vi "ASD total S analysis.vi"(4 "AF_C":cluster{"Anal Time":string, "Filename":string}, 5 "1s datapoint":i32, 6 "Read Region Point":i32=10000, 7 "B Region Time [s] in":dbl, 8 "Rigon#":i32, 9 "Region Count":dbl[](array[numeric]), 10 "Region STD":dbl[](array[numeric]), 11 "Region BL":dbl[](array[numeric])) -> (3 "A Cluster":T1)   [LabVIEW 2018]
uses:
  <vilib>/Analysis/baseanly.llb/Unimode.vi
  <vilib>/Analysis/NI_AALBase.lvlib
panel:
  out "B Duty Cycle [%]":dbl
  out "Total Time [s]":dbl
  out "Region Count Mode":dbl caption="R Count Mode [a]"
  out "Region BL Mode":dbl caption="R BL Mode [pA]"
  out "Region STD Mode":dbl caption="R STD Mode [pA]"
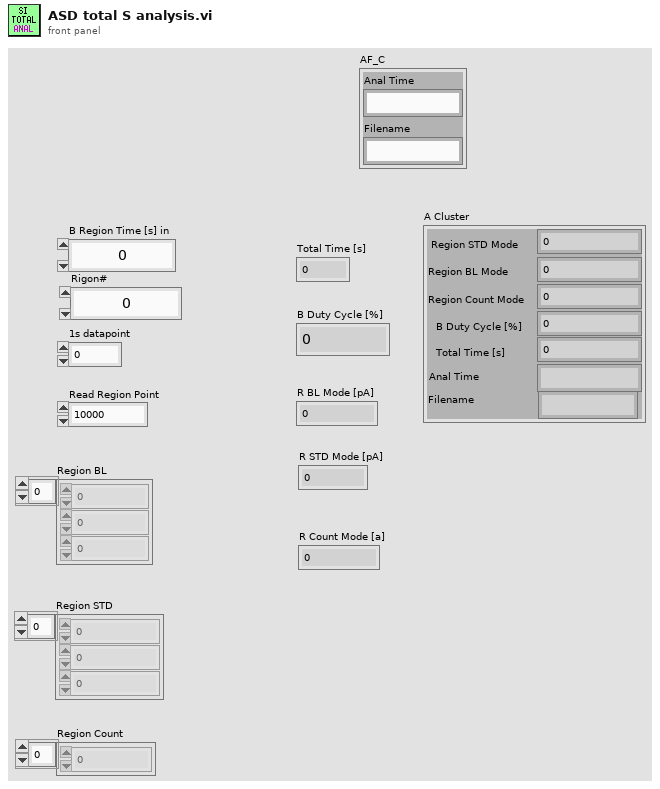
[diagram p1: front panel]
types:
  T1 = cluster{"Region STD Mode":dbl, "Region BL Mode":dbl, "Region Count Mode":dbl, "B Duty Cycle [%]":dbl, "Total Time [s]":dbl, "Anal Time":string, "Filename":string}
  T2 = cluster{"mode":dbl, "mode":dbl, "mode":dbl, dbl, dbl, "Anal Time":string, "Filename":string}
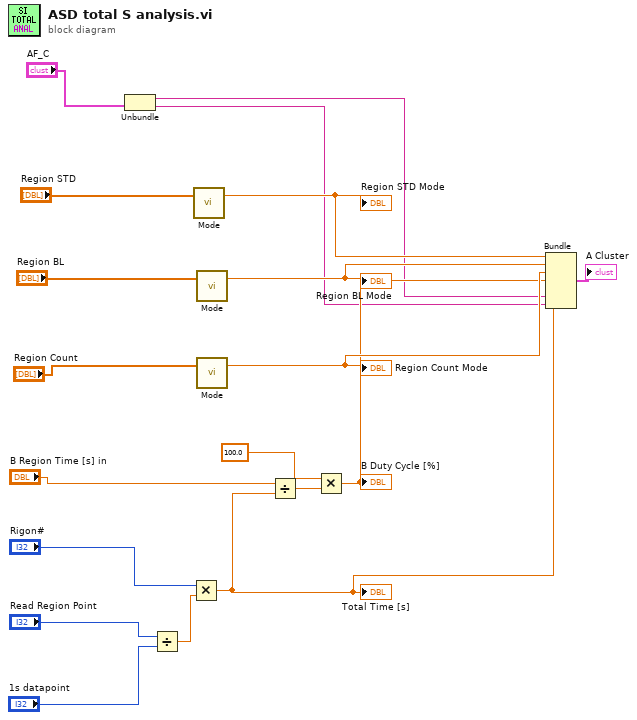
[diagram p0: block diagram]
diagram:
  n1 = Unbundle("AF_C") -> ("Anal Time"=w3:string, "Filename"=w2:string)
  n2 = Divide(x="Read Region Point", y="1s datapoint") -> (x/y=w13:dbl)
  n3 = Multiply(x="Rigon#", y=w13) -> (x*y=w4:dbl)
  "Total Time [s]" <- w4
  n4 = call-poly <vilib>:"Mode.vi"("X"="Region STD") -> ("mode"=w8:dbl)  [unwired: 1 in, 1 out]
  "Region STD Mode" <- w8
  n5 = call-poly <vilib>:"Mode.vi"("X"="Region BL") -> ("mode"=w7:dbl)  [unwired: 1 in, 1 out]
  "Region BL Mode" <- w7
  n6 = call-poly <vilib>:"Mode.vi"("X"="Region Count") -> ("mode"=w6:dbl)  [unwired: 1 in, 1 out]
  "Region Count Mode" <- w6
  n7 = Divide(x="B Region Time [s] in", y=w4) -> (x/y=w11:dbl)
  n8 = Multiply(x=100.0, y=w11) -> (x*y=w5:dbl)
  "B Duty Cycle [%]" <- w5
  n9 = Bundle("mode"=w8, "mode"=w7, "mode"=w6, w5, w4, "Anal Time"=w3, "Filename"=w2) -> (→"A Cluster":T2)  [unwired: 1 in]
